vi "test-simpleSpreadsheet.vi"() -> ()   [LabVIEW 2009]
uses:
  <vilib>/Utility/sysdir.llb/System Directory Type.ctl
  ooCalc/ooCalc.lvclass
panel:
  in  "cell 2":cluster{"Row":u32, "Column":u32}={"Row"=3, "Column"=2}
  in  "cell 1":cluster{"Row":u32, "Column":u32}={"Row"=2, "Column"=3}
  out "Calc error":errorcluster
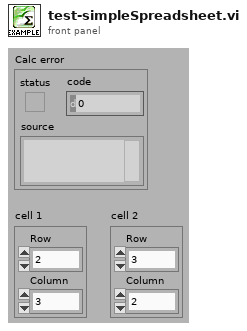
[diagram p1: front panel]
types:
  T1 = typedef "System Directory Type.ctl" = i32
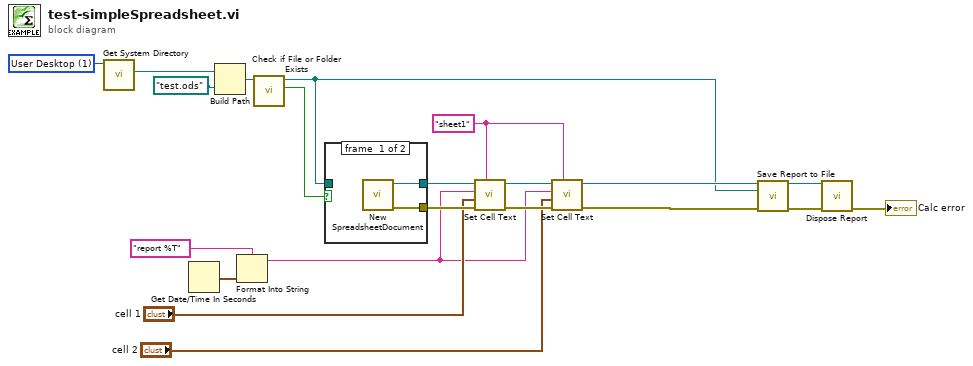
[diagram p0: block diagram]
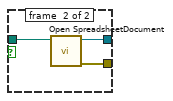
[diagram p2: hidden frame]
diagram:
  w13 = "sheet1" ("Sheet Name")
  w21 = T1 1 items=["User Home", "User Desktop", "User Documents", "User Application Data", "User Preferences", "User Temporary", "Public Documents", "Public Application Data", "Public Preferences", "System Core Libraries", "System Installed Libraries", "Application Files", "Boot Volume Root"] ("system directory type")
  n1 = call <vilib>:"Get System Directory.vi"("system directory type"=w21) -> ("system directory"=w20:path)  [unwired: 10 in]
  n2 = Get Date/Time In Seconds() -> (seconds since 1Jan1904=w3:timestamp)
  n3 = Build Path(base path=w20, name or relative path=path "test.ods") -> (appended path=w6:path)
  n4 = Format Into String(format string="report %T" ("text"), w3) -> (resulting string=w1:string)  [unwired: 2 in, 1 out]
  n5 = call <vilib>:"Check if File or Folder Exists.vi"("path"=w6) -> ("file or folder exists?"=w5:bool, "dup path"=w4:path)  [unwired: 8 in, 1 out]
  n6 = case shown="False" w5 {
    tunnel: [w23 w26] -> w18
    tunnel: [w22 w24] -> w17
    tunnel: w4 -> [_ w25]
    frame #0 {
      n7 = call "New SpreadsheetDocument.vi"() -> ("error out"=w22:errorcluster, "ooCalc out"=w23:refnum<class "ooCalc.lvclass">)  [unwired: 10 in]
    }
    frame #1 {
      n8 = call "Open SpreadsheetDocument.vi"("filepath"=w25) -> ("error out"=w24:errorcluster, "ooCalc out"=w26:refnum<class "ooCalc.lvclass">)  [unwired: 9 in]
    }
  }
  n9 = call-dynamic "Set Cell Text.vi"("Sheet Name"=w13, "error in (no error)"=w17, "position"="cell 1", "text"=w1, "report in"=w18) -> ("error out"=w14:errorcluster, "report out"=w15:refnum<class "ooCalc.lvclass">)  [unwired: 5 in]
  n10 = call-dynamic "Set Cell Text.vi"("Sheet Name"=w13, "error in (no error)"=w14, "position"="cell 2", "text"=w1, "report in"=w15) -> ("error out"=w11:errorcluster, "report out"=w10:refnum<class "ooCalc.lvclass">)  [unwired: 5 in]
  n11 = call-dynamic "Save Report to File.vi"("report in"=w10, "report file path"=w4, "error in (no error)"=w11) -> ("report out"=w9:refnum<class "ooCalc.lvclass">, "error out"=w8:errorcluster)  [unwired: 11 in]
  n12 = call-dynamic "Dispose Report.vi"("report in"=w9, "error in (no error)"=w8) -> ("error out"=→"Calc error":errorcluster)  [unwired: 13 in]
